vi "RT Driver VI.vi"(7 "Operation":T1, 11 "Device Reference in":T2 format="%.0x") -> (0 "Error Code":i32)   [LabVIEW 2025, in "Protection and Counter Addon Engine.lvlib"]
uses:
  Protection and Counter Addon Engine.lvlib
  <vilib>/NI VeriStand/Custom Device API/Custom Device Item Ref.ctl
  <vilib>/NI VeriStand/Custom Device API/Hardware Interface Driver VI Operation.ctl
  <vilib>/NI/NIVS Inline Async API/_VS Inline Async API/VS Inline Async API/Types/Error Handling Settings.ctl
  Addon Shared/Types/Exported.OnCompile.ctl
  Addon Shared/Types/XNET Settings.ctl
  SubModules/Frame-Protection-Support/Source/Shared/Types/Protection Type.ctl
  SubModules/Frame-Protection-Support/Source/Shared/Types/Exported Frame Settings.ctl
  SubModules/Frame-Protection-Support/Source/Shared/Types/Exported Frame Type.ctl
  SubModules/Frame-Protection-Support/Source/Shared/Types/Exported Protection Settings.ctl
  SubModules/Frame-Protection-Support/Source/Shared/Types/XNET Signal Configuration.ctl
  SubModules/Frame-Protection-Support/Source/Shared/Types/Exported Counter Settings.ctl
  SubModules/Frame-Protection-Support/Source/Shared/Types/Exported Event Trigger Type.ctl
  Addon Shared/Types/986x.ctl
  <vilib>/NI/NIVS Inline Async API/_VS Inline Async API/VS Inline Async API/VS Inline Async API.lvclass
  Types/RT Async Engine Settings.ctl
  SubModules/Frame-Protection-Support/Source/Engine/Types/RT Frame Settings.ctl
  SubModules/Frame-Protection-Support/Source/Engine/Types/RT Protection Configuration.ctl
  SubModules/Frame-Protection-Support/Source/Engine/Types/RT Frame Incoming Values.ctl
  <vilib>/NI/NIVS Inline Async API/_VS Inline Async API/VS Inline Async API/VS Inline Async API.lvclass/VS Inline Async API.ctl
  <vilib>/NI/NIVS Inline Async API/_Data Access Engine/Data Access Engine/Data Access Engine.lvclass/Data Access Engine.ctl
  <vilib>/NI/NIVS Inline Async API/_Data Access Engine/Access Type Classes/Write/Write.lvclass/Write.ctl
  <vilib>/NI/NIVS Inline Async API/_Data Access Engine/Access Type Classes/ReadWrite/ReadWrite.lvclass/ReadWrite.ctl
  <vilib>/NI/NIVS Inline Async API/_Data Access Engine/Access Type Classes/Read/Read.lvclass/Read.ctl
  SubVIs/Bitfile.Initialize.vi
  SubModules/Frame-Protection-Support/Source/Engine/SubVIs/Initialize Protection Frames Outgoing.vi
  <vilib>/NI/NIVS Inline Async API/_Data Access Engine/Data Access Engine/Methods/Data.Engine.Read Data from HW.vi
  <vilib>/NI/NIVS Inline Async API/_VS Inline Async API/Error Handling Process/SubVIs/Error.GetError.vi
  <vilib>/NI/NIVS Inline Async API/_Data Access Engine/Data Access Engine/Methods/Data.Engine.Write Data to HW.vi
  SubVIs/Bitfile.Download.vi
  <vilib>/NI/NIVS Inline Async API/_Data Access Engine/Access Type Classes/ReadWrite/ReadWrite.EngineData.vi
  <vilib>/NI/NIVS Inline Async API/_Data Access Engine/Access Type Classes/Write/Write.EngineData.vi
  <vilib>/NI/NIVS Inline Async API/_Data Access Engine/Access Type Classes/Read/Read.EngineData.vi
  <vilib>/NI VeriStand/Custom Device API/NI VeriStand - Get Channel Value by Data Reference.vi
  <vilib>/NI VeriStand/Custom Device API/NI VeriStand - Set Channel Value by Data Reference.vi
  <vilib>/NI VeriStand/Custom Device API/NI VeriStand - Set Channel Values by Block Data Reference.vi
  <vilib>/NI VeriStand/Custom Device API/NI VeriStand - Get Channel Values by Block Data Reference.vi
  Addon Shared/SubVIs/GUID Lookup.vi
  <vilib>/NI VeriStand/Custom Device API/Get Item Property (Variant).vi
  <vilib>/Utility/libraryn.llb/Check if File or Folder Exists.vi
  <vilib>/Utility/error.llb/Error Cluster From Error Code.vi
  <vilib>/rvi/Utilities/XML/nirviXML_GetValue.vi
  <vilib>/rvi/Utilities/XML/nirviXML_GetValue_String.vi
  <vilib>/xnet/xnet.llb/XNET Create Session.vi
  <vilib>/xnet/xnet.llb/XNET Create Session (Frame Output Stream).vi
  <vilib>/xnet/xnet.llb/XNET Create Session (Conversion).vi
  SubModules/Frame-Protection-Support/Source/Engine/SubVIs/Initialize Protection Frames Incoming.vi
  <vilib>/xnet/xnet.llb/XNET Create Session (Frame Input Stream).vi
  <vilib>/Utility/SystemLogging/Write to System Log.vi
  <vilib>/NI VeriStand/Custom Device API/Global Data Refs.vi
  <vilib>/NI VeriStand/Custom Device API/Custom Device API.lvlib
  Addon Shared/Protection and Counter Addon Shared.lvlib
  SubModules/Frame-Protection-Support/Source/Shared/Protection and Counter Support Shared.lvlib
  <vilib>/NI VeriStand/Custom Device Tools/Custom Device Utility Library/Custom Device Utility Library.lvlib
  SubModules/Frame-Protection-Support/Source/Engine/Protection and Counter Support Engine.lvlib
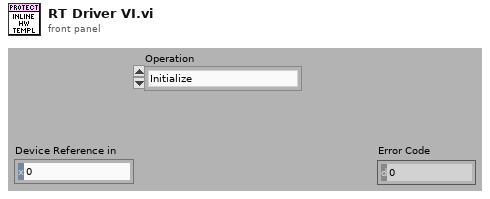
[diagram p1: front panel]
types:
  T1 = typedef "Custom Device API.lvlib/Hardware Interface Driver VI Operation.ctl" = enum16{"Initialize", "Start", "Read Data from HW", "Write Data to HW", "Close"}
  T2 = typedef "Custom Device API.lvlib/Custom Device Item Ref.ctl" = u64
  T3 = typedef "Protection and Counter Addon Engine.lvlib/RT Async Engine Settings.ctl" = cluster{"Name":string, "Priority":i32, "XNET Settings":T4, "FPGA Session":u32, "Outgoing CAN Session":refnum<k21>, "Outgoing Frame Count":i32, "Outgoing Frames":T6[], "Incoming CAN Session":refnum<k21>, "Incoming Frame Count":i32, "Incoming Frames":T6[], "Incoming Values":T12}
  T4 = typedef "Protection and Counter Addon Shared.lvlib/XNET Settings.ctl" = cluster{"Database":refnum<k21>, "Cluster":refnum<k21>, "Port":string, "Baud rate [Bd]":u64, "Termination":u32, "CAN I/O Mode":u32, "FD Baud rate [Bd]":u64, "Priority":i32, "Use Legacy":bool, "FD ISO Mode":u32, "Default Max Counter Value":dbl, "Default Protect Type":T5, "Include All Channels":bool}
  T5 = typedef "Protection and Counter Support Shared.lvlib/Protection Type.ctl" = enum16{"Arb ID + Bytes Checksum with Inversion", "Arb ID + Bytes CRC with Inversion", "Reversed Raw Signal Checksum with Inversion", "Concatenated Two's Compliment"}
  T6 = typedef "Protection and Counter Support Engine.lvlib/RT Frame Settings.ctl" = cluster{"Type":T7, "Frame ID":u32, "Payload Length":u32, "VS Offset":i32, "VS Length":i32, "Frame Conversion":refnum<k21>, "Frame.Data":dbl[], "Generation Period":u32, "Time Since Last Generation":u32, "Generation Iterations":u32, "Generation Counter":u32, "Has Protection?":bool, "Protection Configurations":T8[], "Has Counter?":bool, "Counter Configurations":T10[], "Has Disable?":bool, "Disable VS Index":i32, "Transmit Trigger":T11, "Trigger VS Index":i32}
  T7 = typedef "Protection and Counter Support Shared.lvlib/Exported Frame Type.ctl" = enum16{"Periodic", "Event", "Periodic/Event"}
  T8 = typedef "Protection and Counter Support Engine.lvlib/RT Protection Configuration.ctl" = cluster{"Protection Frame Index":i32, "Protection Type":T5, "Data Indeces":i32[], "Data Array":dbl[], "Check Sum Conversion":refnum<k21>, "CRC Channels":T9[], "Protection VS Index":i32, "Counter Data Index":i32, "Override Index":i32, "Override Value Index":i32}
  T9 = typedef "Protection and Counter Support Shared.lvlib/XNET Signal Configuration.ctl" = cluster{"Start Bit":i32, "Name":string, "Number of bits":i32, "Scale":dbl, "Offset":dbl, "Data Type":u32, "Counter":bool}
  T10 = typedef "Protection and Counter Support Shared.lvlib/Exported Counter Settings.ctl" = cluster{"Frame Index":i32, "Max Count":dbl, "VS Index":i32, "Bit Length":i64, "Override Index":i32, "Override Value Index":i32}
  T11 = typedef "Protection and Counter Support Shared.lvlib/Exported Event Trigger Type.ctl" = enum16{"Channel value change", "Trigger channel (not zero)", "Channel value change or trigger channel (not zero)", "Trigger channel (any value change)", "Channel value change or trigger channel (any value change)"}
  T12 = typedef "Protection and Counter Support Engine.lvlib/RT Frame Incoming Values.ctl" = cluster{"Signal Values":dbl[], "Signal Invalid Values":dbl[], "ProtCtr Sig Values":dbl[], "Timestamps":timestamp[], "Time Differences":dbl[], "IDs":u32[]}
  T13 = cluster{"Process":refnum<class "VS Inline Async API.lvclass">, "RT Configuration":T3}
  T14 = typedef "VS Inline Async API.lvlib/VS Inline Async API.lvclass/Error Handling Settings.ctl" = cluster{"Write to SystemLog (F)":bool}
  T15 = typedef "Protection and Counter Addon Shared.lvlib/Exported.OnCompile.ctl" = cluster{"Name":string, "XNET Settings":T4, "Frames":T16[], "986x Support":T18, "Incoming Frames":T16[]}
  T16 = typedef "Protection and Counter Support Shared.lvlib/Exported Frame Settings.ctl" = cluster{"Type":T7, "Frame ID":u32, "Payload Length":u32, "Signal XNET Paths":string[], "Frame.PrevData":dbl[], "VS Offset":i32, "VS Length":i32, "Generation Period":u32, "Has Protection?":bool, "Protection Configurations":T17[], "Has Counter":bool, "Counter Configurations":T10[], "Has Disable?":bool, "Disable VS Index":i32, "Transmit Trigger":T11, "Trigger VS Index":i32}
  T17 = typedef "Protection and Counter Support Shared.lvlib/Exported Protection Settings.ctl" = cluster{"Protection Frame Index":i32, "Protection Type":T5, "Data Indeces":i32[], "Initialized Data Array":dbl[], "Protection Signal XNET Paths":string[], "CRC Channels":T9[], "Protection VS Update Index":i32, "Override Index":i32, "Override Value Index":i32}
  T18 = typedef "Protection and Counter Addon Shared.lvlib/986x.ctl" = cluster{"Enable":bool, "RIO Device":string, "Bitfile":path}
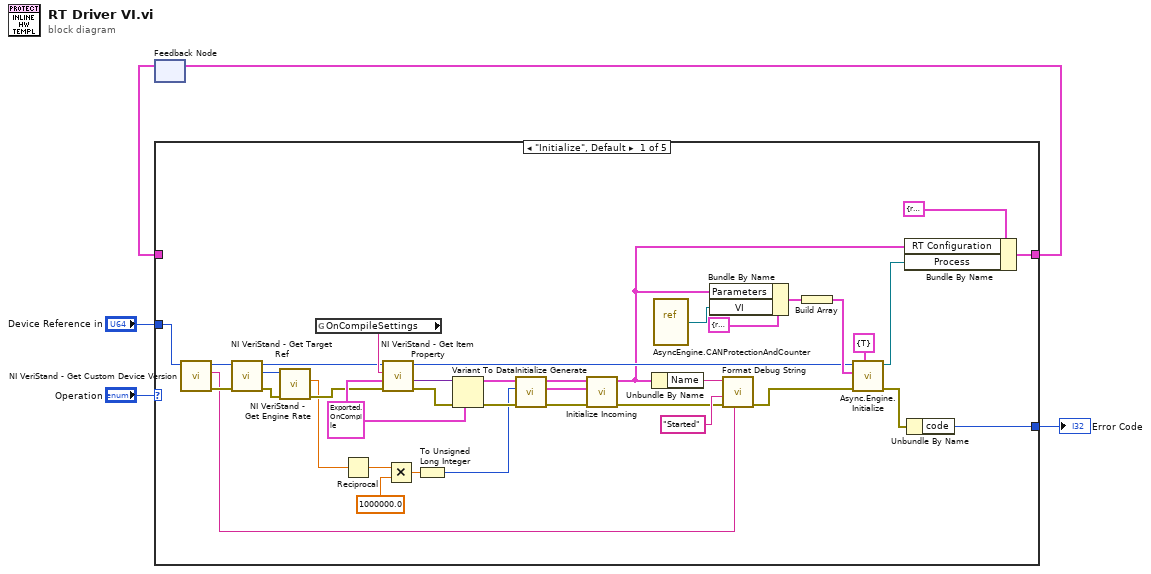
[diagram p0: block diagram]
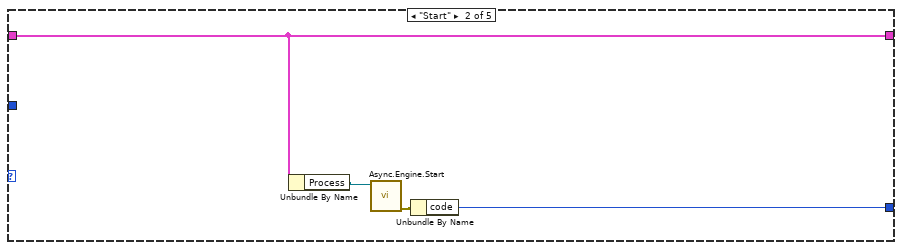
[diagram p2: hidden frame]
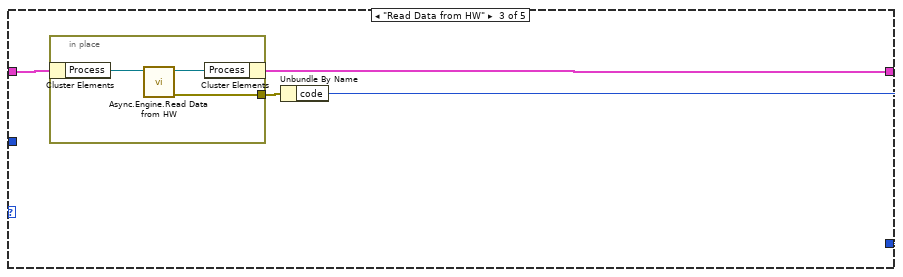
[diagram p3: hidden frame]
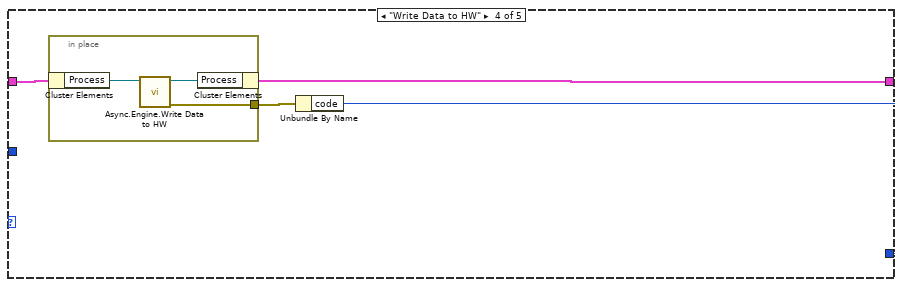
[diagram p4: hidden frame]
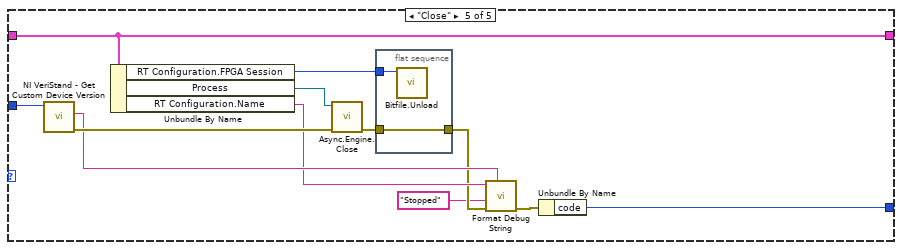
[diagram p5: hidden frame]
diagram:
  n1 = feedback #1() -> (w3:T13)  [unwired: 1 out]
  n2 = case shown="\"Initialize\", Default" "Operation" {
    tunnel: [w42 w44 w50 w58 w70] -> w4
    tunnel: w3 -> [_ w44 w51 w57 w70]
    tunnel: [w43 w47 w48 w55 w65] -> w2
    tunnel: "Device Reference in" -> [w41 _ _ _ w73]
    frame "Initialize", Default {
      w31 = T15 {"Name"="", "XNET Settings"={"Database"="", "Cluster"="", "Port"="", "Baud rate [Bd]"=500000, "Termination"=1, "CAN I/O Mode"=0, "FD Baud rate [Bd]"=500000, "Priority"=100, "Use Legacy"=FALSE, "FD ISO Mode"=0, "Default Max Counter Value"=0.0, "Default Protect Type"=enum."Arb ID + Bytes Checksum with Inversion", "Include All Channels"=FALSE}, "Frames"=[], "986x Support"={"Enable"=FALSE, "RIO Device"="", "Bitfile"=path ""}, "Incoming Frames"=[]} ("Cluster")
      n3 = call <vilib>:"NI VeriStand - Get Custom Device Version.vi"("Device Ref in"=w41) -> ("error out"=w25:errorcluster, "Value"=w14:string, "Device Ref out"=w34:T2)  [unwired: 8 in]
      n4 = call <vilib>:"NI VeriStand - Get Target Ref.vi"("error in"=w25, "Item Ref in"=w34) -> ("error out"=w24:errorcluster, "Target Ref"=w26:T2, "Item Ref out"=w27:T2)  [unwired: 6 in, 1 out]
      n5 = call <vilib>:"NI VeriStand - Get Engine Rate.vi"("error in (no error)"=w24, "Item Ref in"=w26) -> ("error out"=w23:errorcluster, "Rate (Hz)"=w22:dbl)  [unwired: 7 in, 1 out]
      n6 = global read "GUID Lookup.vi" "OnCompileSettings"() -> (w35:string)
      n7 = Reciprocal(x=w22) -> (1/x=w21:dbl)
      n8 = call-poly <vilib>:"NI VeriStand - Get Item Property.vi"("error in (no error)"=w23, "Default Value"=w31, "Property Name"=w35, "Item Ref in"=w27) -> ("error out"=w32:errorcluster, "Value"=w33:variant, "Item Ref out"=w30:T2)  [unwired: 4 in, 1 out]
      n9 = Multiply(x=w21, y=1000000.0) -> (x*y=w19:dbl)
      n10 = To Unsigned Long Integer(number=w19) -> (unsigned 32bit integer=w18:u32)
      n11 = Variant To Data(error in=w32, type=w31, Variant=w33) -> (data=w11:T15, error out=w29:errorcluster)
      n12 = call "Initialize Generate.vi"("error in (no error)"=w29, "PCL (usec)"=w18, "OnCompile Variables"=w11) -> ("error out"=w10:errorcluster, "RT Configuration"=w7:T3, "OnCompile Variables out"=w6:T15)  [unwired: 6 in]
      n13 = call "Initialize Incoming.vi"("error in (no error)"=w10, "RT Configuration In"=w7, "OnCompile Variables"=w6) -> ("error out"=w9:errorcluster, "RT Configuration Out"=w8:T3)  [unwired: 7 in]
      n14 = Unbundle By Name(w8) -> ("Name"=w16:string)
      n15 = vi-ref "AsyncEngine.CANProtectionAndCounter.vi"() -> (w28:refnum<vi>)
      n16 = Bundle By Name(cluster=cluster{"VI":refnum<vi>, "Parameters":variant} {"VI"=refnum, "Parameters"=variant} ("Process"), "Parameters"=w8, "VI"=w28) -> (w38:cluster{"VI":refnum<vi>, "Parameters":variant})
      n17 = call "Format Debug String.vi"("Version"=w14, "error in (no error)"=w9, "State"="Started", "Name"=w16) -> ("error out"=w12:errorcluster)  [unwired: 7 in]
      n18 = Build Array(w38) -> (w37:cluster{"VI":refnum<vi>, "Parameters":variant}[])
      n19 = call <vilib>:"Async.Engine.Initialize.vi"("Error Log Settings"=T14 {"Write to SystemLog (F)"=TRUE}, "error in (no error)"=w12, "Processes"=w37, "Custom Device Ref"=w30) -> ("error out"=w13:errorcluster, "Async"=w40:refnum<class "VS Inline Async API.lvclass">)  [unwired: 6 in]
      n20 = Bundle By Name(cluster=T13 {"Process"=refnum, "RT Configuration"={"Name"="", "Priority"=100, "XNET Settings"={"Database"="", "Cluster"="", "Port"="", "Baud rate [Bd]"=0, "Termination"=0, "CAN I/O Mode"=0, "FD Baud rate [Bd]"=500000, "Priority"=100, "Use Legacy"=FALSE, "FD ISO Mode"=0, "Default Max Counter Value"=0.0, "Default Protect Type"=enum."Arb ID + Bytes Checksum with Inversion", "Include All Channels"=FALSE}, "FPGA Session"=0, "Outgoing CAN Session"="", "Outgoing Frame Count"=0, "Outgoing Frames"=[], "Incoming CAN Session"="", "Incoming Frame Count"=0, "Incoming Frames"=[], "Incoming Values"={"Signal Values"=[], "Signal Invalid Values"=[], "ProtCtr Sig Values"=[], "Timestamps"=[], "Time Differences"=[], "IDs"=[]}}} ("input cluster"), "RT Configuration"=w8, "Process"=w40) -> (w42:T13)
      n21 = Unbundle By Name(w13) -> ("code"=w43:i32)
    }
    frame "Start" {
      n22 = Unbundle By Name(w44) -> ("Process"=w46:refnum<class "VS Inline Async API.lvclass">)
      n23 = call <vilib>:"Async.Engine.Start.vi"("VS Inline Async API in"=w46) -> ("error out"=w45:errorcluster)  [unwired: 9 in, 1 out]
      n24 = Unbundle By Name(w45) -> ("code"=w47:i32)
    }
    frame "Read Data from HW" {
      n25 = in-place {
        in-place-border: [w52] -> w49
        n26 = in-place-cluster #2(w51) -> ("Process"=w54:refnum<class "VS Inline Async API.lvclass">)
        n27 = call <vilib>:"Async.Engine.Read Data from HW.vi"("Async in"=w54) -> ("error out"=w52:errorcluster, "Async out"=w53:refnum<class "VS Inline Async API.lvclass">)  [unwired: 9 in]
        n28 = in-place-cluster #2("Process"=w53) -> (w50:T13)
      }
      n29 = Unbundle By Name(w49) -> ("code"=w48:i32)
    }
    frame "Write Data to HW" {
      n30 = in-place {
        in-place-border: [w59] -> w56
        n31 = in-place-cluster #3(w57) -> ("Process"=w61:refnum<class "VS Inline Async API.lvclass">)
        n32 = call <vilib>:"Async.Engine.Write Data to HW.vi"("VS Inline Async API in"=w61) -> ("error out"=w59:errorcluster, "VS Inline Async API out"=w60:refnum<class "VS Inline Async API.lvclass">)  [unwired: 9 in]
        n33 = in-place-cluster #3("Process"=w60) -> (w58:T13)
      }
      n34 = Unbundle By Name(w56) -> ("code"=w55:i32)
    }
    frame "Close" {
      n35 = call <vilib>:"NI VeriStand - Get Custom Device Version.vi"("Device Ref in"=w73) -> ("error out"=w69:errorcluster, "Value"=w68:string)  [unwired: 8 in, 1 out]
      n36 = Unbundle By Name(w70) -> ("RT Configuration.FPGA Session"=w71:u32, "Process"=w72:refnum<class "VS Inline Async API.lvclass">, "RT Configuration.Name"=w67:string)
      n37 = call <vilib>:"Async.Engine.Close.vi"("error in (no error)"=w69, "Async in"=w72) -> ("error out"=w62:errorcluster)  [unwired: 8 in, 1 out]
      n38 = flat-sequence {
        tunnel: w71 -> [w75]
        tunnel: w62 -> [w74]
        tunnel: [w74] -> w66
        frame #0 {
          n39 = call "Bitfile.Unload.vi"("Session"=w75) -> ()  [unwired: 11 in]
        }
      }
      n40 = call "Format Debug String.vi"("Version"=w68, "error in (no error)"=w66, "State"="Stopped", "Name"=w67) -> ("error out"=w63:errorcluster)  [unwired: 7 in]
      n41 = Unbundle By Name(w63) -> ("code"=w65:i32)
    }
  }
  "Error Code" <- w2
  n42 = feedback-in #1(w4) -> ()
